vi "libssh2_sftp_last_error.vi"(8 "error in (no error)":errorcluster, 11 "sftp":T1) -> (0 "error out":errorcluster)   [LabVIEW 2017, in "libssh2.lvlib"]
doc: "Get the last error code and error message for an SFTP session.\n\nThis only works when libssh2 returned <B>LIBSSH2_ERROR_SFTP_PROTOCOL</B> in a previous call. Otherwise, the return value is undefined."
uses:
  libssh2.lvlib
  SFTP Refnum.ctl
  Acquire Session.vi
  Release Session.vi
  Global Settings.vi
  Read SFTP Refnum.vi
  Read Session Refnum.vi
  <vilib>/Utility/semaphor.llb/Acquire Semaphore.vi
  <vilib>/Utility/semaphor.llb/Release Semaphore.vi
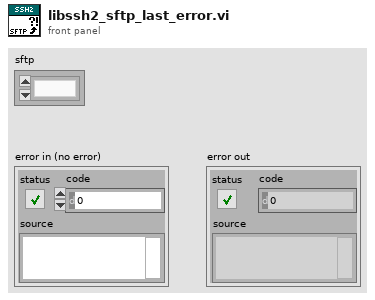
[diagram p1: front panel]
types:
  T1 = typedef "libssh2.lvlib/SFTP Refnum.ctl" = refnum<k1>
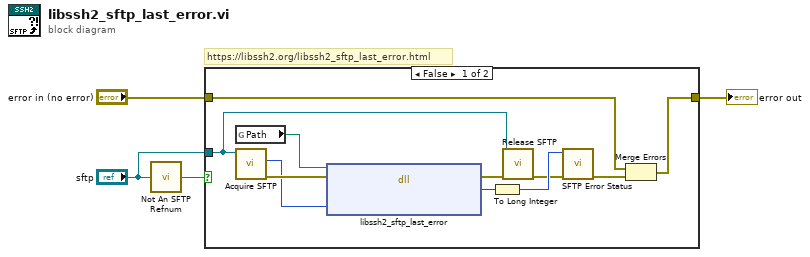
[diagram p0: block diagram]
diagram:
  # "https://libssh2.org/libssh2_sftp_last_error.html"
  n1 = call "Not An SFTP Refnum.vi"("sftp"="sftp") -> ("Not a SFTP Refnum?"=w4:bool)
  n2 = case shown="False" w4 {
    tunnel: "sftp" -> [w5 _]
    tunnel: [w8 w16] -> w3
    tunnel: "error in (no error)" -> [w10 w16]
    frame False {
      n3 = global read "Global Settings.vi" "Path"() -> (w15:path)
      n4 = call "Acquire SFTP.vi"("sftp"=w5) -> ("error out"=w14:errorcluster, "LIBSSH2_SFTP*"=w13:u64)  [unwired: 9 in]
      n5 = dll-call lib="?" fn="libssh2_sftp_last_error"(path in=w15, error in=w14, "sftp"=w13) -> (error out=w12:errorcluster, "return value"=w11:u32)  [unwired: 2 in, 1 out]
      n6 = To Long Integer(number=w11) -> (32bit integer=w7:i32)
      n7 = call "Release SFTP.vi"("error in (no error)"=w12, "sftp"=w5) -> ("error out"=w6:errorcluster)  [unwired: 9 in]
      n8 = call "SFTP Error Status.vi"("error in (no error)"=w6, "return value"=w7) -> ("error out"=w9:errorcluster)  [unwired: 8 in, 1 out]
      n9 = Merge Errors(w10, w9) -> (w8:errorcluster)
    }
    frame True {
    }
  }
  "error out" <- w3
